vi "Import and Export Controls.vi"() -> ()   [LabVIEW 2013, in "DCAF UI Elements.lvlib"]
uses:
  Controls/DCAF UI Elements.lvlib
  Controls/Import.ctl
  Controls/Export.ctl
panel:
  in  "Export":T1
  in  "Import":T2
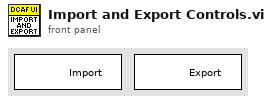
[diagram p1: front panel]
types:
  T1 = typedef "DCAF UI Elements.lvlib/Export.ctl" = bool
  T2 = typedef "DCAF UI Elements.lvlib/Import.ctl" = bool
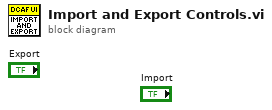
[diagram p0: block diagram]
diagram:
